vi "Auto Scroll Tree.vi"(8 "error in":errorcluster, 10 "TreeControl in":refnum<vi>, 11 "Recent root tags IN":string[](array[string])) -> (0 "error out":errorcluster, 3 "Recent root tags OUT":string[](array[string]))   [LabVIEW 2025, in "CAN-LIN Raw Bus Capture UI.lvlib"]
doc: "This VI creates a buffer, and checks if the buffer size is more then 19, then it deletes the oldest element, adds the new one to the end, and sets the TREE's top left cell to the oldest one. So the latest 20 element will be shown in the tree."
uses:
  CAN-LIN Raw Bus Capture UI.lvlib
  <vilib>/Utility/miscctls.llb/LVNodeAndColumnTypeDef.ctl
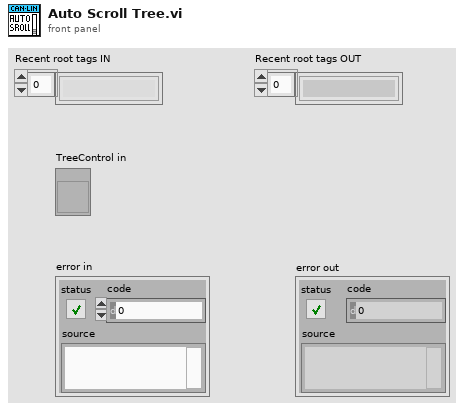
[diagram p1: front panel]
types:
  T1 = typedef "LVNodeAndColumnTypeDef.ctl" = cluster{"Node":string, "Column":i32}
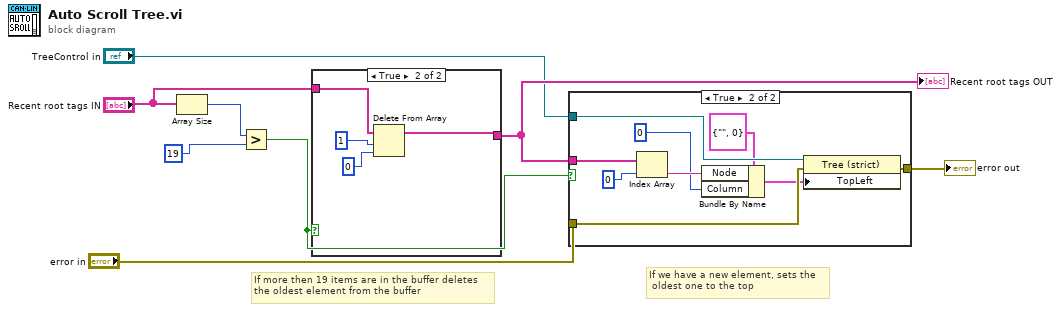
[diagram p0: block diagram]
diagram:
  # "If we have a new element, sets the\n oldest one to the top"
  # "If more then 19 items are in the buffer deletes\nthe oldest element from the buffer"
  n1 = Array Size(array="Recent root tags IN") -> (size(s)=w7:i32)
  n2 = Greater?(x=w7, y=19) -> (0:w2:bool)
  n3 = case shown="True" w2 {
    tunnel: "Recent root tags IN" -> [w9 w10]
    tunnel: [w9 w11] -> w4
    frame False {
    }
    frame True {
      n4 = Delete From Array(array=w10, length=1, index=0) -> (array with subset deleted=w11:string[])  [unwired: 1 out]
    }
  }
  "Recent root tags OUT" <- w4
  n5 = case shown="True" w2 {
    tunnel: [w14 w23] -> w8
    tunnel: w4 -> [_ w22]
    tunnel: "TreeControl in" -> [_ w19]
    tunnel: "error in" -> [w14 w18]
    frame False {
    }
    frame True {
      n6 = Index Array(array=w22, index=0) -> (element=w20:string)
      n7 = Bundle By Name(cluster=T1 {"Node"="", "Column"=0} ("Top Left Visible Cell"), "Node"=w20, "Column"=0) -> (w15:T1)
      n8 = property class="Tree (strict)"(reference=w19, error in=w18, "TopLeft"=w15) -> (error out=w23:errorcluster)  [unwired: 1 out]
    }
  }
  "error out" <- w8
